vi "DSS-Tests-summary_array.vi"(11 "values":dbl[](array[numeric])) -> (3 "summary":dbl[](array[numeric]))   [LabVIEW 2020, in "DSS-Tests.lvlib"]
doc: "Summarises a 1D DBL array as three values: its length, its first element and its last element (0 for an empty array)."
uses:
  DSS-Tests.lvlib
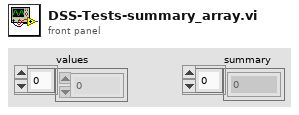
[diagram p1: front panel]
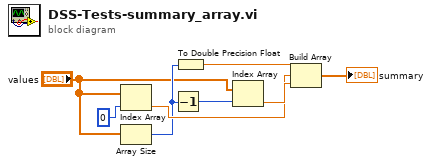
[diagram p0: block diagram]
diagram:
  n1 = Index Array(array="values", index=0 ("first index")) -> (element=w6:dbl)
  n2 = Array Size(array="values") -> (size(s)=w2:i32)
  n3 = Decrement(x=w2) -> (x-1=w4:i32)
  n4 = To Double Precision Float(number=w2) -> (double precision float=w3:dbl)
  n5 = Index Array(array="values", index=w4) -> (element=w7:dbl)
  n6 = Build Array(w3, w6, w7) -> (→"summary":dbl[])
